vi "Generate Getter VI.vi"(7 "Highlight changes?":bool=TRUE, 8 "error in (no error)":errorcluster, 9 "class path":path, 10 "Attribute Name":string) -> (0 "error out":errorcluster)   [LabVIEW 2020, in "Method Generation.lvlib" / "Getter Generator.lvclass"]
uses:
  Getter Generator.lvclass
  Getter Generator.lvclass/Getter Generator.ctl
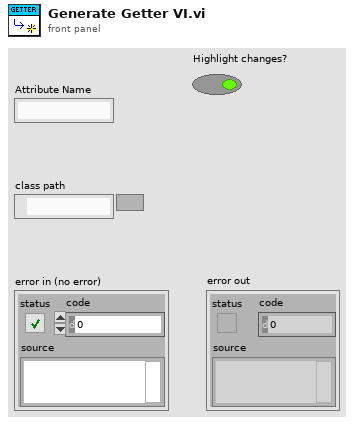
[diagram p1: front panel]
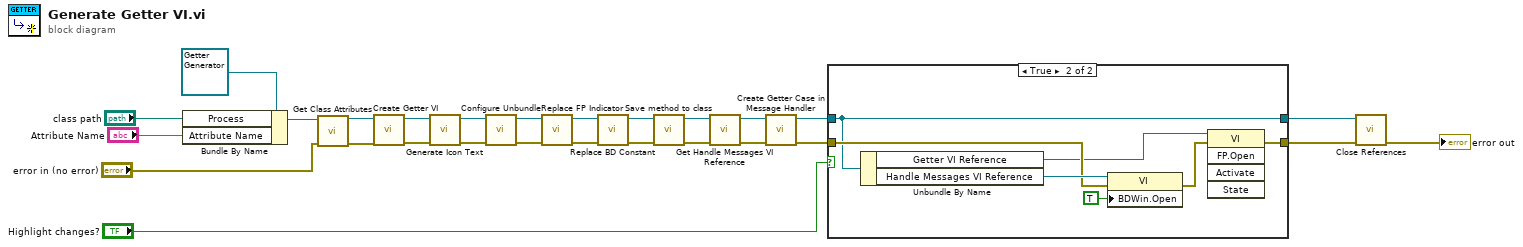
[diagram p0: block diagram]
diagram:
  n1 = Bundle By Name(cluster=refnum<class "Getter Generator.lvclass"> refnum ("New Getter Dialog In"), "Process"="class path", "Attribute Name"="Attribute Name") -> (w19:refnum<class "Getter Generator.lvclass">)
  n2 = call "Get Class Attributes.vi"("error in (no error)"="error in (no error)", "New Getter Dialog In"=w19) -> ("error out"=w23:errorcluster, "New Getter Dialog Out"=w22:refnum<class "Getter Generator.lvclass">)  [unwired: 8 in]
  n3 = call "Create Getter VI.vi"("error in (no error)"=w23, "New Getter Dialog in"=w22) -> ("error out"=w25:errorcluster, "New Getter Dialog out"=w2:refnum<class "Getter Generator.lvclass">)  [unwired: 8 in]
  n4 = call "Generate Icon Text.vi"("error in (no error)"=w25, "Getter Generator in"=w2) -> ("error out"=w3:errorcluster, "Getter Generator out"=w1:refnum<class "Getter Generator.lvclass">)  [unwired: 8 in]
  n5 = call "Configure Unbundle.vi"("error in (no error)"=w3, "Getter Generator in"=w1) -> ("error out"=w17:errorcluster, "Getter Generator out"=w26:refnum<class "Getter Generator.lvclass">)  [unwired: 8 in]
  n6 = call "Replace FP Indicator.vi"("error in (no error)"=w17, "Getter Generator In"=w26) -> ("error out"=w16:errorcluster, "Getter Generator Out"=w27:refnum<class "Getter Generator.lvclass">)  [unwired: 8 in]
  n7 = call "Replace BD Constant.vi"("error in (no error)"=w16, "Getter Generator In"=w27) -> ("error out"=w14:errorcluster, "Getter Generator Out"=w13:refnum<class "Getter Generator.lvclass">)  [unwired: 8 in]
  n8 = call "Save method to class.vi"("error in (no error)"=w14, "Getter Generator In"=w13) -> ("error out"=w10:errorcluster, "Getter Generator Out"=w11:refnum<class "Getter Generator.lvclass">)  [unwired: 8 in]
  n9 = call "Get Handle Messages VI Reference.vi"("error in (no error)"=w10, "Getter Generator in"=w11) -> ("error out"=w12:errorcluster, "Getter Generator out"=w9:refnum<class "Getter Generator.lvclass">)  [unwired: 8 in]
  n10 = call "Create Getter Case in Message Handler.vi"("error in (no error)"=w12, "Getter Generator in"=w9) -> ("error out"=w8:errorcluster, "Getter Generator out"=w5:refnum<class "Getter Generator.lvclass">)  [unwired: 8 in]
  n11 = case shown="True" "Highlight changes?" {
    tunnel: w5 -> [w28 w30]
    tunnel: w8 -> [w29 w34]
    tunnel: [w29 w32] -> w7
    tunnel: [w28 w30] -> w4
    frame False {
    }
    frame True {
      n12 = Unbundle By Name(w30) -> ("Getter VI Reference"=w31:refnum<vi>, "Handle Messages VI Reference"=w36:refnum<vi>)
      n13 = property class="VI"(reference=w36, error in=w34, "BDWin.Open"=TRUE ("Block Diagram Window:Open")) -> (error out=w33:errorcluster)  [unwired: 1 out]
      n14 = invoke class="VI" method="FP.Open"(reference=w31, error in=w33) -> (error out=w32:errorcluster)  [unwired: 3 in, 4 out]
    }
  }
  n15 = call "Close References.vi"("error in (no error)"=w7, "Getter Generator in"=w4) -> ("error out"=→"error out":errorcluster)  [unwired: 9 in]
